vi "Edit Line.vi"(8 "error in":errorcluster, 10 "Line Name":string, 11 "References":T1) -> (0 "error out":errorcluster, 2 "change?":bool)   [LabVIEW 2015, in "DAQmx Module editor node.lvclass"]
doc: "This VI edits the properties of a line. It will unlink channels and tags and create new links to channels and tags."
uses:
  DAQmx Module editor node.lvclass
  <vilib>/NI/DCAF/Tag Editor Core/Table API/Table Manager/object ref.ctl
  <vilib>/NI/DCAF/Tag Editor Core/Configuration Editor/Classes/Engine Parent/Engine Parent Editor Node.lvclass
  <vilib>/NI/DCAF/Tag Editor Core/Configuration Editor/Classes/Module editor node/module editor node.lvclass
  module/configuration/Daqmx Module configuration.lvclass
  module/configuration/Daqmx Module configuration.lvclass/Daqmx Module configuration.ctl
  <vilib>/NI/Configuration Framework/serializable configuration/NISE_CEF_serializable configuration.lvclass/NISE_CEF_serializable configuration.ctl
  <vilib>/Utility/LVClass/Get LV Class Name.vi
  <vilib>/NI/Configuration Framework/error generator/NISE_error generator.vi
  <vilib>/NI/Tag Bus Module Framework/channel/TBM channel.lvclass
  <vilib>/NI/Configuration Framework/serializable configuration/NISE_CEF_serializable configuration.lvclass
  <vilib>/NI/DCAF/Tag Editor Core/Table API/Table Manager/Table Manager.lvclass
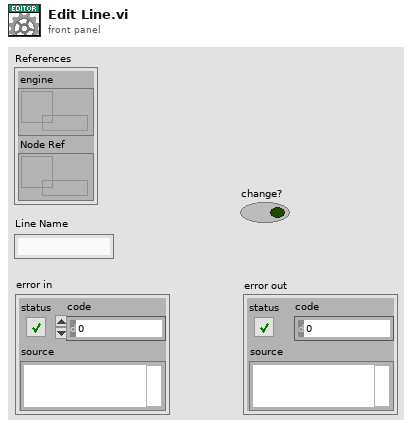
[diagram p1: front panel]
types:
  T1 = typedef "Table Manager.lvlib/Table Manager.lvclass/object ref.ctl" = cluster{"engine":refnum<data-value>, "Node Ref":refnum<data-value>}
  T2 = typedef "DAQmx Module Configuration.lvclass/Line.ctl" = cluster{"Channel Array":refnum<class "TBM channel.lvclass">[], "Physical Channel":string, "Measurement Type":T3, "Parameters":T4}
  T3 = typedef "DAQmx Module Configuration.lvclass/Measurement Type.ctl" = enum16{"Digital Input", "Digital Output", "Voltage Input", "Voltage Output", "Current Input", "Current Output", "RTD", "Thermocouple", "Strain", "PWM"}
  T4 = typedef "DAQmx Module Configuration.lvclass/Parameters.ctl" = cluster{"Digital Config":cluster{"Invert Lines?":bool}, "Voltage Config":cluster{"Maximum Value (V)":dbl, "Minimum Value (V)":dbl, "in terminal configuration (V)":i32, "out terminal configuration (V)":i32}, "Current Config":cluster{"Maximum Value (A)":dbl, "Minimum Value (A)":dbl, "shunt resistor location":i32, "input terminal configuration (C)":i32, "external shunt resistor value":dbl}, "RTD Config":cluster{"Maximum Value (°C)":dbl, "Minimum Value (°C)":dbl, "resistance configuration":i32, "r0":dbl, "current excitation value":dbl, "rtd type":i32, "current excitation source":i32}, "Thermocouple Config":cluster{"Minimum Value (C)":dbl, "Maximum Value (C)":dbl, "thermocouple type":i32, "cjc source":i32, "cjc value":dbl}, "Strain Config":cluster{"Maximum Value":dbl, "Minimum Value":dbl, "bridge information":cluster{"strain configuration":i32, "lead wire resistance":dbl, "initial bridge voltage":dbl, "voltage excitation source":i32, "voltage excitation value":dbl}, "strain gage information":cluster{"gage factor":dbl, "nominal gage resistance":dbl, "poisson ratio":dbl}}, "PWM Config":cluster{"Idle State":bool}}
  T5 = typedef "DAQmx Module editor node.lvclass/Mappings.ctl" = cluster{"Line":T2, "Maps":T6[]}
  T6 = typedef "DAQmx Module editor node.lvclass/Map.ctl" = cluster{"channel":refnum<class "TBM channel.lvclass">, "tag name":string}
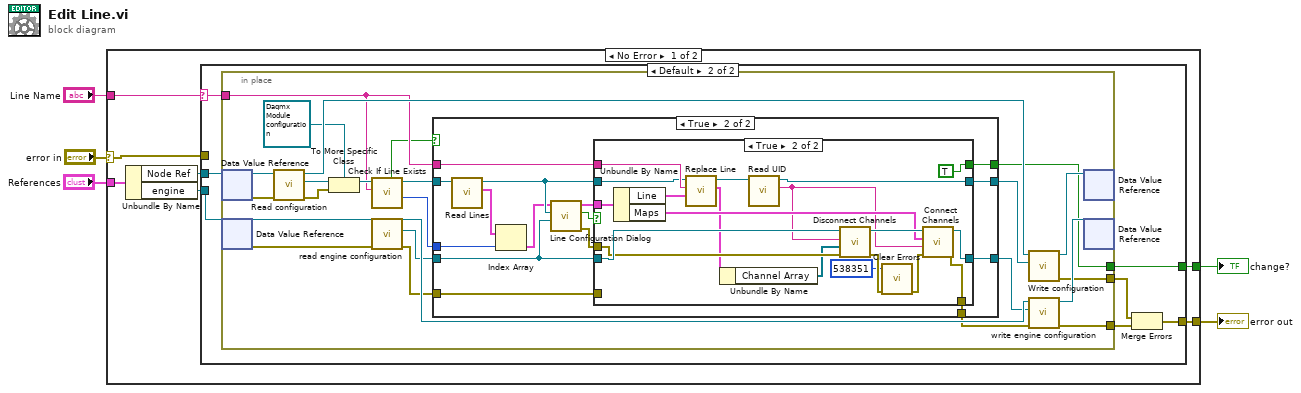
[diagram p0: block diagram]
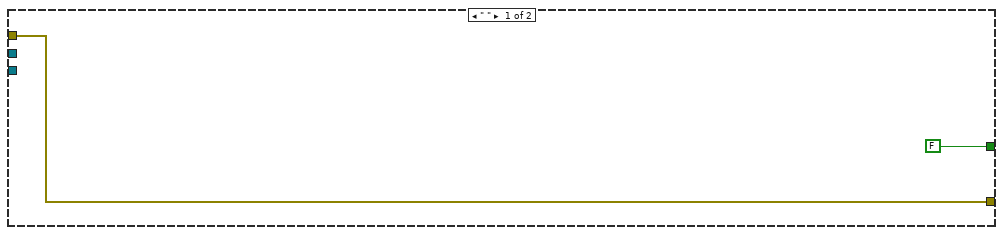
[diagram p2: hidden frame]
diagram:
  n1 = case shown="No Error" "error in" {
    selector: "error in" -> [w6 w86]
    tunnel: "References" -> [w10 _]
    tunnel: "Line Name" -> [w7 _]
    tunnel: [w9 w86] -> w2
    tunnel: [w8 _] -> w1
    frame No Error {
      n2 = Unbundle By Name(w10) -> ("Node Ref"=w12:refnum<data-value>, "engine"=w11:refnum<data-value>)
      n3 = case shown="Default" w7 {
        selector: w7 -> [_ w15]
        tunnel: w12 -> [_ w21]
        tunnel: w11 -> [_ w20]
        tunnel: [w13 w17] -> w9
        tunnel: [FALSE ("change?") w16] -> w8
        tunnel: w6 -> [w13 _]
        frame " " {
        }
        frame Default {
          n4 = in-place {
            in-place-border: [w27] -> w19
            in-place-border: [w42] -> w18
            in-place-border: [w26] -> w16
            in-place-border: w15 -> [w32]
            n5 = in-place-dvr #1(w21) -> (w39:refnum<class "module editor node.lvclass">, w33:errorcluster)
            n6 = in-place-dvr #2(w20) -> (w45:refnum<class "Engine Parent Editor Node.lvclass">, w44:errorcluster)
            n7 = call-dynamic "Read configuration.vi"("error in"=w33, "NISE_CEF_serializable node in"=w39) -> ("error out"=w36:errorcluster, "configuration"=w37:refnum<class "NISE_CEF_serializable configuration.lvclass">, "NISE_CEF_serializable node out"=w38:refnum<class "module editor node.lvclass">)  [unwired: 7 in]
            n8 = To More Specific Class(target class=refnum<class "Daqmx Module configuration.lvclass"> refnum ("tag bus configurable plugin module configuration"), reference=w37, error in=w36) -> (specific class reference=w34:refnum<class "Daqmx Module configuration.lvclass">)  [unwired: 1 out]
            n9 = call-dynamic "Check If Line Exists.vi"("Name to Locate"=w32, "Daqmx Module configuration in"=w34) -> ("Index"=w29:i32, "Daqmx Module configuration out"=w30:refnum<class "Daqmx Module configuration.lvclass">, "Found?"=w24:bool)  [unwired: 5 in, 2 out]
            n10 = call <vilib>:"read engine configuration.vi"("error in"=w44, "Engine Parent Editor Node in"=w45) -> ("error out"=w22:errorcluster, "engine configuration"=w28:refnum<class "engine configuration.lvclass">, "Engine Parent Editor Node out"=w41:refnum<class "Engine Parent Editor Node.lvclass">)  [unwired: 7 in]
            n11 = case shown="True" w24 {
              tunnel: w30 -> [w48 w61]
              tunnel: w28 -> [w47 w52]
              tunnel: w32 -> [_ w63]
              tunnel: [w48 w56] -> w31
              tunnel: w29 -> [_ w58]
              tunnel: [_ w54] -> w26
              tunnel: [w47 w53] -> w25
              tunnel: [w46 w50] -> w23
              tunnel: w22 -> [w46 w49]
              frame False {
              }
              frame True {
                n12 = call "Read Lines.vi"("Daqmx Module configuration in"=w61) -> ("Lines"=w59:T2[], "Daqmx Module configuration out"=w60:refnum<class "Daqmx Module configuration.lvclass">)  [unwired: 8 in, 1 out]
                n13 = Index Array(array=w59, index=w58) -> (element=w51:T2)
                n14 = call "Line Configuration Dialog.vi"("engine configuration in"=w52, "tag bus configurable plugin module configuration"=w60, "Line"=w51) -> ("error out"=w62:errorcluster, "changed"=w55:bool, "Mappings out"=w57:T5)  [unwired: 5 in, 1 out]
                n15 = case shown="True" w55 {
                  tunnel: w63 -> [_ w85]
                  tunnel: w52 -> [w65 w84]
                  tunnel: w62 -> [_ w83]
                  tunnel: w60 -> [w66 w81]
                  tunnel: w57 -> [_ w80]
                  tunnel: [w66 w78] -> w56
                  tunnel: [_ TRUE ("change?")] -> w54
                  tunnel: [w65 w73] -> w53
                  tunnel: [w64 w72] -> w50
                  tunnel: w49 -> [w64 _]
                  frame False {
                  }
                  frame True {
                    n16 = Unbundle By Name(w80) -> ("Line"=w79:T2, "Maps"=w76:T6[])
                    n17 = call "Replace Line.vi"("New Line"=w79, "Line Name"=w85, "Daqmx Module configuration in"=w81) -> ("Old Line"=w67:T2, "Daqmx Module configuration out"=w82:refnum<class "Daqmx Module configuration.lvclass">)  [unwired: 6 in, 1 out]
                    n18 = Unbundle By Name(w67) -> ("Channel Array"=w68:refnum<class "TBM channel.lvclass">[])
                    n19 = call <vilib>:"Read UID.vi"("configuration in"=w82) -> ("instance id"=w75:string, "configuration out"=w78:refnum<class "Daqmx Module configuration.lvclass">)  [unwired: 8 in, 1 out]
                    n20 = call "Disconnect Channels.vi"("error in (no error)"=w83, "Deleted Channels"=w68, "instance id"=w75, "Engine Configuration in"=w84) -> ("error out"=w71:errorcluster, "Engine Configuration out"=w77:refnum<class "engine configuration.lvclass">)  [unwired: 6 in]
                    n21 = call <vilib>:"Clear Errors.vi"("error in (no error)"=w71, "specific error code to clear (0: all)"=538351) -> ("error out"=w70:errorcluster)  [unwired: 4 in, 1 out]
                    n22 = call "Connect Channels.vi"("error in (no error)"=w70, "instance id"=w75, "Maps"=w76, "Engine Configuration in"=w77) -> ("error out"=w72:errorcluster, "Engine Configuration out"=w73:refnum<class "engine configuration.lvclass">)  [unwired: 6 in]
                  }
                }
              }
            }
            n23 = call-dynamic "Write configuration.vi"("configuration"=w31, "NISE_CEF_serializable node in"=w38) -> ("error out"=w27:errorcluster, "NISE_CEF_serializable node out"=w40:refnum<class "module editor node.lvclass">)  [unwired: 8 in]
            n24 = call <vilib>:"write engine configuration.vi"("error in"=w23, "engine configuration"=w25, "Engine Parent Editor Node in"=w41) -> ("error out"=w42:errorcluster, "Engine Parent Editor Node out"=w43:refnum<class "Engine Parent Editor Node.lvclass">)  [unwired: 7 in]
            n25 = in-place-dvr #1(w40) -> ()  [unwired: 2 out]
            n26 = in-place-dvr #2(w43) -> ()  [unwired: 2 out]
          }
          n27 = Merge Errors(w19, w18) -> (w17:errorcluster)
        }
      }
    }
    frame Error {
    }
  }
  "change?" <- w1
  "error out" <- w2
